vi "Get Control From Type Descriptor__A2E.vi"(0 "VI Refnum":refnum<vi>, 1 "error in (no error)":errorcluster, 2 "data type":variant) -> (3 "VI Refnum":refnum<vi>, 4 "New Control Ref":refnum<vi>, 5 "error out":errorcluster)   [LabVIEW 2021, in "Utilities.lvlib"]
uses:
  Utilities.lvlib
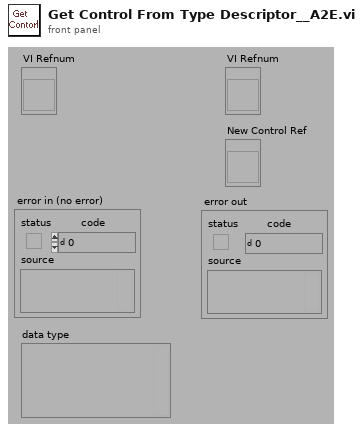
[diagram p1: front panel]
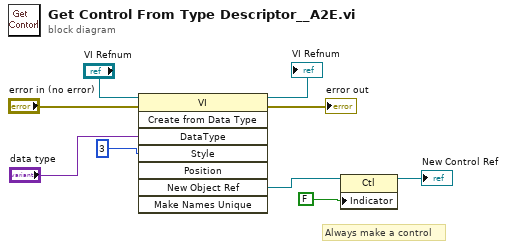
[diagram p0: block diagram]
diagram:
  # "Always make a control"
  n1 = invoke class="VI" method="Create from Data Type"(reference="VI Refnum", error in="error in (no error)", "DataType"="data type", "Style"=3 ("style")) -> (reference out=→"VI Refnum":refnum<vi>, error out=→"error out":errorcluster, "New Object Ref"=w2:refnum<vi>)  [unwired: 4 in, 5 out]
  n2 = property class="Ctl"(reference=w2, "Indicator"=FALSE) -> (reference out=→"New Control Ref":refnum<vi>)  [unwired: 1 in, 1 out]
